vi "Read pathname.vi"(8 "error in (no error)":errorcluster, 11 "Unix Pipe in":refnum<class "Unix Pipe.lvclass">) -> (0 "error out":errorcluster, 2 "pathname":string, 3 "Unix Pipe out":refnum<class "Unix Pipe.lvclass">)   [LabVIEW 2016, in "Linux RT IPC.Pipes.lvlib" / "Unix Pipe.lvclass"]
uses:
  Unix Pipe.lvclass
  Unix Pipe.lvclass/Unix Pipe.ctl
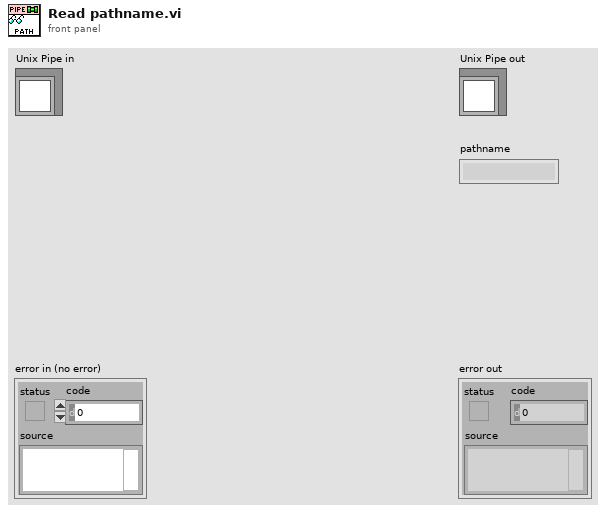
[diagram p1: front panel]
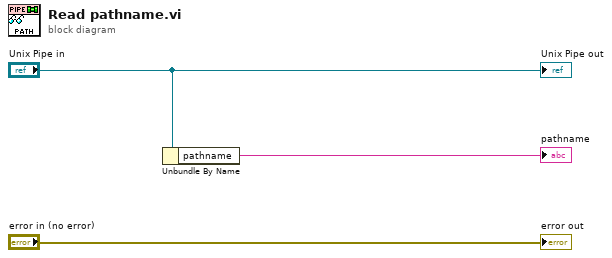
[diagram p0: block diagram]
diagram:
  n1 = Unbundle By Name("Unix Pipe in") -> ("pathname"=→"pathname":string)
  "error out" <- "error in (no error)"
  "Unix Pipe out" <- "Unix Pipe in"
